vi "PSK Modulator.vi"(0 "Baseband Signal":dbl[](array[numeric]), 1 "Sampling Frequency(Fs)":dbl, 2 "Carrier Frequency (fc)":dbl, 3 "Carrier Amplitude (A)":dbl, 4 "Phase for Binary 1":dbl=3.14159) -> (5 "PSK Modulated Waveform":dbl[](array[numeric]))   [LabVIEW 2026]
panel:
  out "PSK Modulated Waveform":dbl[](graph)
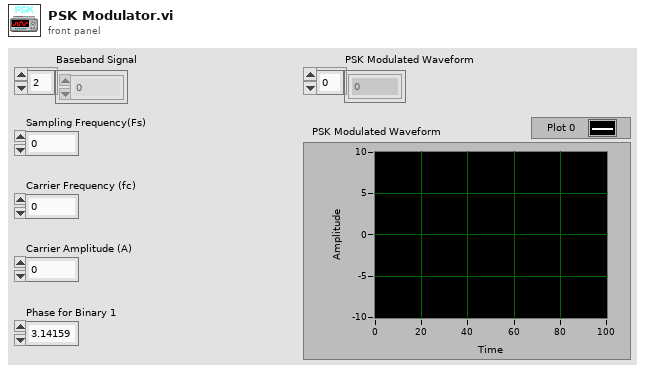
[diagram p1: front panel]
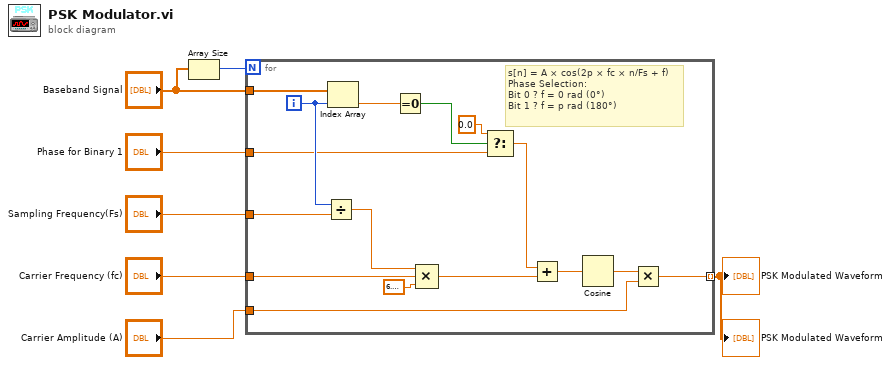
[diagram p0: block diagram]
diagram:
  n1 = Array Size(array="Baseband Signal") -> (size(s)=w7:i32)
  n2 = for {
    N: w7 -> [_]
    tunnel: "Baseband Signal" -> [w23]
    tunnel: "Sampling Frequency(Fs)" -> [w21]
    tunnel: "Carrier Frequency (fc)" -> [w19]
    tunnel: "Phase for Binary 1" -> [w15]
    tunnel: "Carrier Amplitude (A)" -> [w9]
    tunnel: [w8] -> w1 mode=indexing
    i -> [w22]
    # "s[n] = A × cos(2p × fc × n/Fs + f)\nPhase Selection:\nBit 0 ? f = 0 rad (0°)\nBit 1 ? f = p rad (180°)"
    n3 = Divide(x=w22, y=w21) -> (x/y=w20:dbl)
    n4 = Index Array(array=w23, index=w22) -> (element=w17:dbl)
    n5 = Equal To 0?(x=w17) -> (x = 0?=w16:bool)
    n6 = Compound Arithmetic op=MULTIPLY(w20, w19, 6.283185307179586) -> (w13:dbl)
    n7 = Select(t=0.0, s=w16, f=w15) -> (s? t:f=w12:dbl)
    n8 = Add(x=w12, y=w13) -> (x+y=w11:dbl)
    n9 = Cosine(x=w11) -> (cos(x)=w10:dbl)
    n10 = Multiply(x=w10, y=w9) -> (x*y=w8:dbl)
  }
  "PSK Modulated Waveform" <- w1
  "PSK Modulated Waveform" <- w1
